vi "Build VIH Deploy - Copy Other Files.vi"(8 "error in":errorcluster, 9 "Files to Copy":path[](array[path]), 10 "Source Dir":path, 11 "Target Dir":path) -> (0 "error out":errorcluster, 3 "dup Target Dir":path)   [LabVIEW 2014]
doc: "::: VI Helpeks :::\nCopyright (c) 2000-2026 Konstantin Shifershteyn. All rights reserved."
panel:
  # "VI Helpeks\nCopyright (c) 2012-2026 Konstantin Shifershteyn"
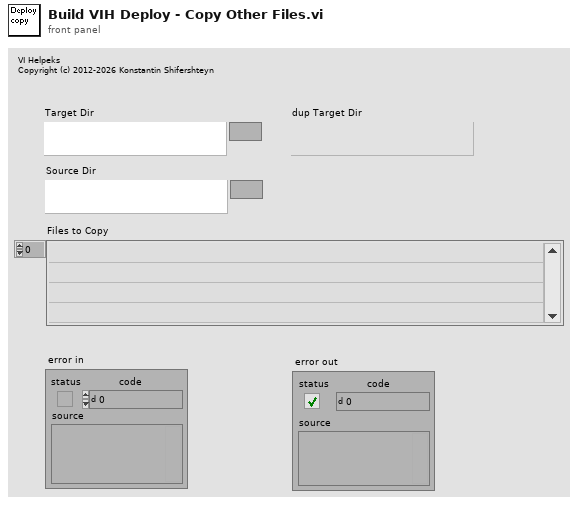
[diagram p1: front panel]
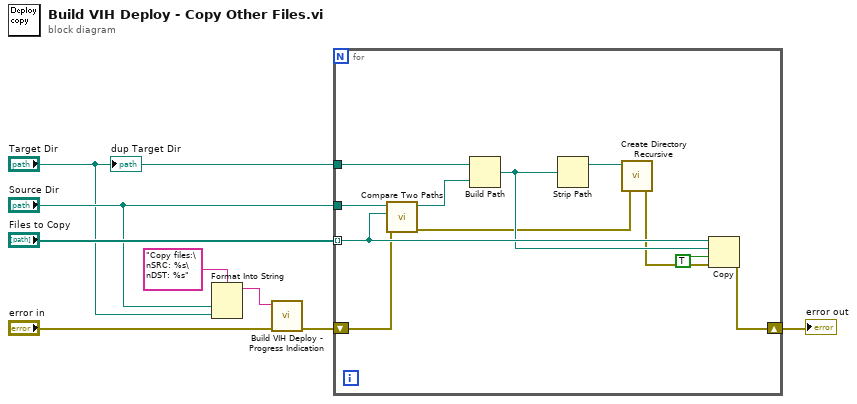
[diagram p0: block diagram]
diagram:
  n1 = Format Into String(format string="Copy files:\nSRC: %s\nDST: %s", "Source Dir", "Target Dir") -> (resulting string=w3:string)  [unwired: 2 in, 1 out]
  n2 = call "Build VIH Deploy - Progress Indication.vi"("error in"="error in", "message 1"=w3) -> ("error out"=w5:errorcluster)  [unwired: 9 in]
  n3 = for {
    tunnel: "Files to Copy" -> [w16] mode=indexing
    tunnel: "Source Dir" -> [w19]
    tunnel: "Target Dir" -> [w18]
    shift-right: [w9] -> w7
    shift-left: w5 -> [w12]
    n4 = call <vilib>:"Compare Two Paths.vi"("error in (no error)"=w12, "Path 2"=w16, "Path 1"=w19) -> ("error out"=w11:errorcluster, "Relative Path from 1 to 2"=w17:path)  [unwired: 5 in, 2 out]
    n5 = Build Path(base path=w18, name or relative path=w17) -> (appended path=w15:path)
    n6 = Strip Path(path=w15) -> (stripped path=w13:path)  [unwired: 1 out]
    n7 = call <vilib>:"Create Directory Recursive.vi"("error in (no error)"=w11, "directory"=w13) -> ("error out"=w10:errorcluster)  [unwired: 3 in, 2 out]
    n8 = Copy(8:w10, 9:TRUE, 10:w15, 11:w16) -> (0:w9:errorcluster)  [unwired: 1 in, 2 out]
  }
  "error out" <- w7
  "dup Target Dir" <- "Target Dir"
